vi "Add File.vi"(8 "error in":errorcluster, 9 "File Path":path, 10 "Whitelist constant":path, 11 "Hash Whitelist Handler in":refnum<class "Hash Whitelist Handler.lvclass">) -> (0 "error out":errorcluster, 3 "Hash Whitelist Handler out":refnum<class "Hash Whitelist Handler.lvclass">)   [LabVIEW 2026, in "Hash Whitelist Handler.lvclass"]
doc: "Add the hash of the provided file to the whitelist constant."
uses:
  Hash Whitelist Handler.lvclass
  Hash Whitelist Handler.lvclass/Hash Whitelist Handler.ctl
  <vilib>/security/Message Digest/API/NI_Message Digest API.lvlib
  <vilib>/security/Message Digest/API/Instances/File/SHA-512 File Checksum.vi
  Interfaces/ILogger/ILogger Messages/Log Msg/Log Msg.lvclass
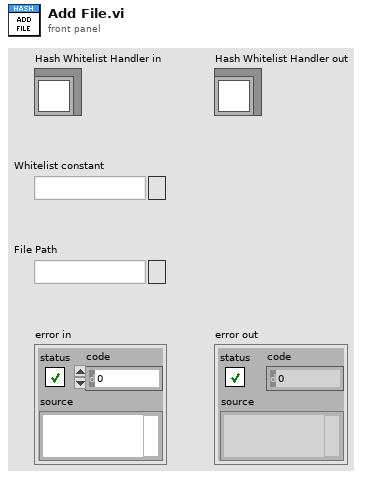
[diagram p1: front panel]
types:
  T1 = typedef "Log Entry--cluster.ctl" = cluster{"Time":timestamp, "Message":string}
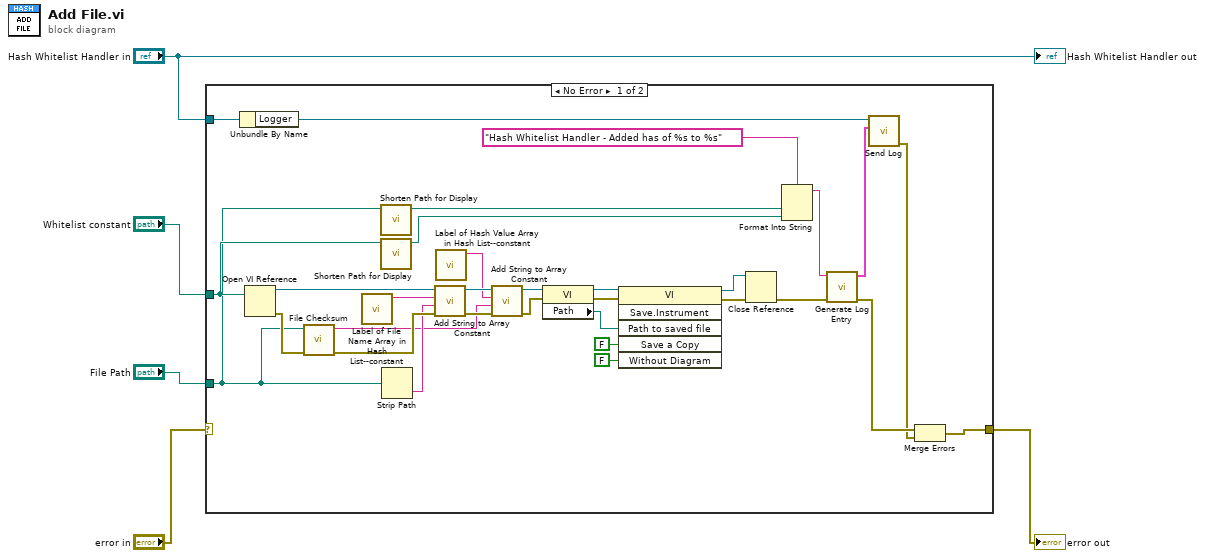
[diagram p0: block diagram]
diagram:
  n1 = case shown="No Error" "error in" {
    selector: "error in" -> [_ w37]
    tunnel: "File Path" -> [w9 _]
    tunnel: [w28 w37] -> w4
    tunnel: "Whitelist constant" -> [w10 _]
    tunnel: "Hash Whitelist Handler in" -> [w14 _]
    frame No Error {
      n2 = Unbundle By Name(w14) -> ("Logger"=w13:refnum<class "Message Enqueuer.lvclass">)
      n3 = Open VI Reference(vi path=w10) -> (vi reference=w26:refnum<vi>, error out=w36:errorcluster)  [unwired: 5 in]
      n4 = call-poly <vilib>:"File Checksum.vi"("error in"=w36, "path"=w9) -> ("error out"=w35:errorcluster, "digest"=w23:string)  [unwired: 8 in]
      n5 = call "Label of File Name Array in Hash List--constant.vi"() -> ("Label of File Name Array in Hash List"=w16:string)  [unwired: 11 in]
      n6 = call "Shorten Path for Display.vi"("Path"=w9) -> ("Shortened Path"=w8:path)  [unwired: 10 in]
      n7 = call "Shorten Path for Display.vi"("Path"=w10) -> ("Shortened Path"=w6:path)  [unwired: 10 in]
      n8 = Strip Path(path=w9) -> (name=w25:string)  [unwired: 1 out]
      n9 = call "Add String to Array Constant.vi"("error in"=w35, "New Value"=w25, "Array Constant Label"=w16, "VI Ref in"=w26) -> ("error out"=w34:errorcluster, "VI Ref out"=w24:refnum<vi>)  [unwired: 6 in]
      n10 = call "Label of Hash Value Array in Hash List--constant.vi"() -> ("Label of File Name Array in Hash List"=w15:string)  [unwired: 11 in]
      n11 = call "Add String to Array Constant.vi"("error in"=w34, "New Value"=w23, "Array Constant Label"=w15, "VI Ref in"=w24) -> ("error out"=w33:errorcluster, "VI Ref out"=w22:refnum<vi>)  [unwired: 6 in]
      n12 = property on="Property Node" class="VI"(reference=w22, error in=w33) -> (reference out=w21:refnum<vi>, error out=w32:errorcluster, "Path"=w20:path)
      n13 = invoke on="Invoke Node" class="VI" method="Save.Instrument"(reference=w21, error in=w32, "Path to saved file"=w20, "Save a Copy"=FALSE, "Without Diagram"=FALSE) -> (reference out=w17:refnum<vi>, error out=w31:errorcluster)  [unwired: 1 in, 4 out]
      n14 = Close Reference(reference=w17, error in (no error)=w31) -> (error out=w30:errorcluster)
      n15 = Format Into String(format string="Hash Whitelist Handler - Added has of %s to %s", w8, w6) -> (resulting string=w7:string)  [unwired: 2 in, 1 out]
      n16 = call "Generate Log Entry.vi"("error in"=w30, "Message"=w7) -> ("error out"=w29:errorcluster, "Log Entry"=w12:T1)  [unwired: 8 in]
      n17 = call "Send Log.vi"("Log Entry"=w12, "Message Enqueuer"=w13) -> ("error out"=w27:errorcluster)  [unwired: 8 in, 1 out]
      n18 = Merge Errors(w29, w27) -> (w28:errorcluster)
    }
    frame Error {
      # "Pass error without further actions."
    }
  }
  "error out" <- w4
  "Hash Whitelist Handler out" <- "Hash Whitelist Handler in"
